vi "GetElements(Multiple).vi"(7 "Qualified Name":string, 8 "error in (no error)":errorcluster, 10 "keys":string[](array[string]), 11 "ConfigManagerCollection in":refnum<class "ConfigManagerCollection.lvclass">) -> (0 "error out":errorcluster, 1 "Values":string[](array[string]), 2 "Keys":string[](array[string]), 3 "ConfigManagerCollection out":refnum<class "ConfigManagerCollection.lvclass">, 4 "Found":bool[](array[boolean]))   [LabVIEW 2013, in "CfgManager.lvlib" / "ConfigManagerCollection.lvclass"]
uses:
  ConfigManagerCollection.lvclass
  Manager/ConfigManager.lvclass
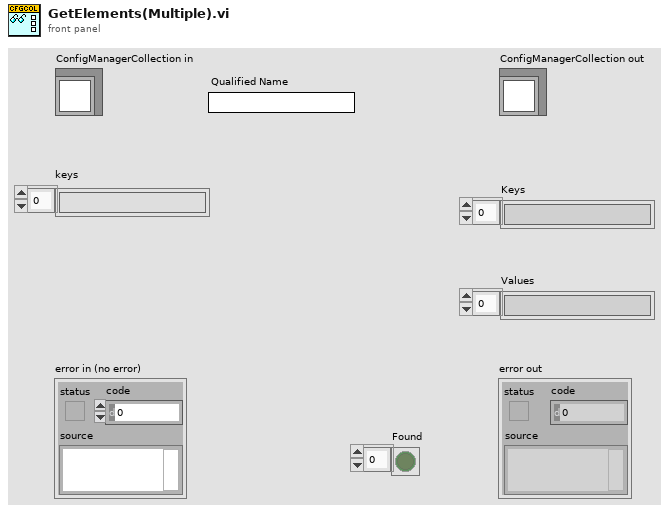
[diagram p1: front panel]
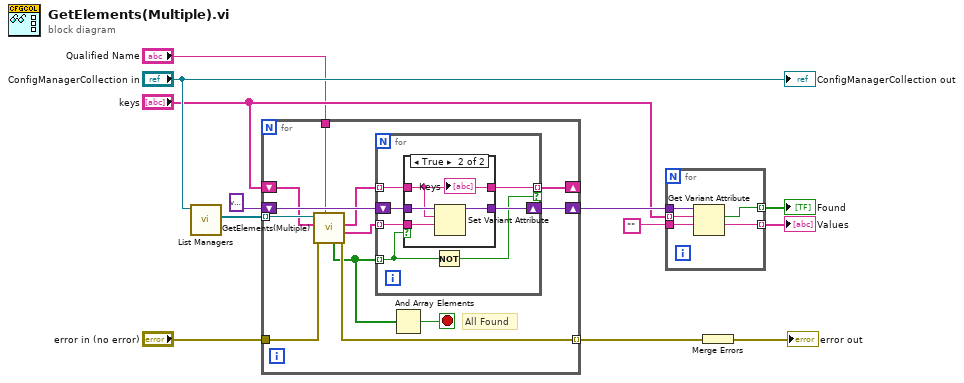
[diagram p0: block diagram]
diagram:
  n1 = call-dynamic "List Managers.vi"("ConfigManagerCollection in"="ConfigManagerCollection in") -> ("List"=w12:refnum<class "ConfigManager.lvclass">[])  [unwired: 9 in, 1 out]
  n2 = for {
    tunnel: w12 -> [w24] mode=indexing
    tunnel: "error in (no error)" -> [w22]
    tunnel: [w21] -> w11 mode=indexing
    shift-right: [w19] -> w6
    shift-left: variant ("variant") -> [w20]
    shift-right: [w18] -> _
    shift-left: "keys" -> [w14]
    tunnel: "Qualified Name" -> [w17]
    stop <- w23 stop-if-true
    # "All Found"
    n3 = call-dynamic "GetElements(Multiple).vi"("Qualified Name"=w17, "error in (no error)"=w22, "keys"=w14, "ConfigManager in"=w24) -> ("error out"=w21:errorcluster, "Values"=w15:string[], "Keys"=w13:string[], "Found"=w16:bool[])  [unwired: 3 in, 1 out]
    n4 = for {
      tunnel: w16 -> [w26] mode=indexing
      shift-right: [w31] -> w19
      shift-left: w20 -> [w30]
      tunnel: w13 -> [w29] mode=indexing
      tunnel: w15 -> [w28] mode=indexing
      tunnel: [w27] -> w18 mode=indexing if=w25
      n5 = case shown="True" w26 {
        tunnel: [w33 w35] -> w31
        tunnel: w30 -> [w33 w36]
        tunnel: w29 -> [w32 w34]
        tunnel: w28 -> [_ w37]
        tunnel: [w32 w34] -> w27
        frame False {
        }
        frame True {
          n6 = Set Variant Attribute(Variant=w36, name=w34, value=w37) -> (Variant out=w35:variant)  [unwired: 1 in, 2 out]
        }
      }
      n7 = Not(x=w26) -> (.not. x?=w25:bool)
    }
    n8 = And Array Elements(Boolean array=w16) -> (logical AND=w23:bool)
  }
  n9 = for {
    tunnel: w6 -> [w42]
    tunnel: "keys" -> [w41] mode=indexing
    tunnel: "" -> [w40]
    tunnel: [w39] -> w3 mode=indexing
    tunnel: [w38] -> w2 mode=indexing
    n10 = Get Variant Attribute(Variant=w42, name=w41, default value (empty Variant)=w40) -> (found=w38:bool, value=w39:string)  [unwired: 1 in, 2 out]
  }
  "Values" <- w3
  "Found" <- w2
  n11 = Merge Errors(w11) -> (→"error out":errorcluster)
  "ConfigManagerCollection out" <- "ConfigManagerCollection in"
